vi "Event_Probe.vi"(11 "OpenLvVision_OpenCv.lvlib:Cuda.lvlib:Event":refnum<class "Event.lvclass">) -> (2 "Value String":string, 3 "Pause VI":bool)   [LabVIEW 2020, in "OpenLvVision_OpenCv.lvlib" / "Cuda.lvlib" / "Event.lvclass"]
uses:
  Event.lvclass
  _LvHelpers/EdvrObject/EdvrObject.lvclass
  C:/Users/lukas/Downloads/OpenLvVision_OpenCv/SourceCode/LabView/OpenLvVision_OpenCv/_LvHelpers/EdvrObject/EdvrObject.lvclass
  C:/Users/lukas/Downloads/OpenLvVision_OpenCv/SourceCode/LabView/OpenLvVision_OpenCv/Cuda/DataAccess/Event/Event.lvclass
panel:
  out "Complete":bool
  out "Reference":u64 format="%.0x"
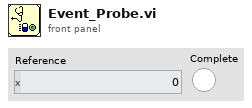
[diagram p1: front panel]
types:
  T1 = typedef "OpenLvVision_OpenCv.lvlib/EdvrObject.lvclass/Edvr.ctl" = refnum<data-value>
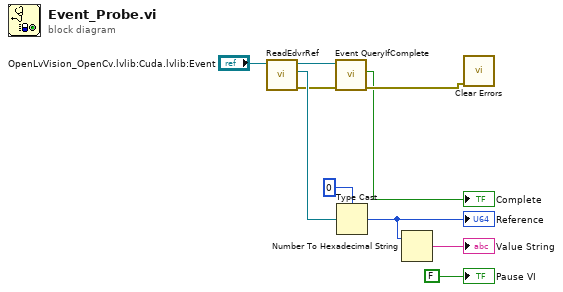
[diagram p0: block diagram]
diagram:
  n1 = call "ReadEdvrRef.vi"("EdvrObject in"="OpenLvVision_OpenCv.lvlib:Cuda.lvlib:Event") -> ("error out"=w3:errorcluster, "Edvr"=w6:T1, "EdvrObject out"=w4:refnum<class "Event.lvclass">)  [unwired: 8 in]
  n2 = call "Event QueryIfComplete.vi"("error in (no error)"=w3, "Event in"=w4) -> ("error out"=w2:errorcluster, "IsComplete?"=→"Complete":bool)  [unwired: 7 in, 1 out]
  n3 = Type Cast(type=u64 0, x=w6) -> (*(type *) &x=w8:u64)
  "Reference" <- w8
  n4 = Number To Hexadecimal String(2:w8) -> (0:→"Value String":string)  [unwired: 1 in]
  n5 = call <vilib>:"Clear Errors.vi"("error in (no error)"=w2) -> ()  [unwired: 5 in, 2 out]
  "Pause VI" <- FALSE
